vi "Parse Structures.vi"(8 "error in":errorcluster, 11 "ParseGDSII in":refnum<class "ParseGDSII.lvclass">) -> (0 "error out":errorcluster, 2 "Geometric":refnum<class "Geometric.lvclass">[](array[class]), 3 "ParseGDSII out":refnum<class "ParseGDSII.lvclass">)   [LabVIEW 2019, in "ParseGDSII.lvclass"]
uses:
  ParseGDSII.lvclass
  Elements/Geometric.lvclass
  ParseGDSII.lvclass/ParseGDSII.ctl
  Fast Tree/Fast Tree.lvclass
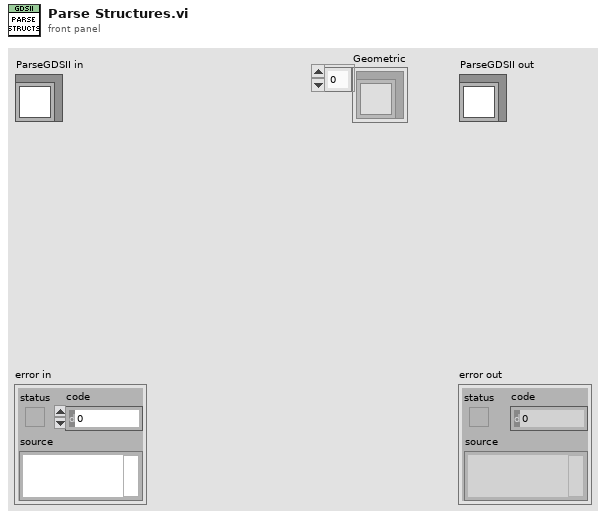
[diagram p1: front panel]
types:
  T1 = cluster{"Record Type":string, "Payload":string, "Parent Index":i32, "First Child Index":i32, "Next Sibling Index":i32}[]
  T2 = cluster{"Record Type":string, "Payload":string, "Parent Index":i32, "First Child Index":i32, "Next Sibling Index":i32}
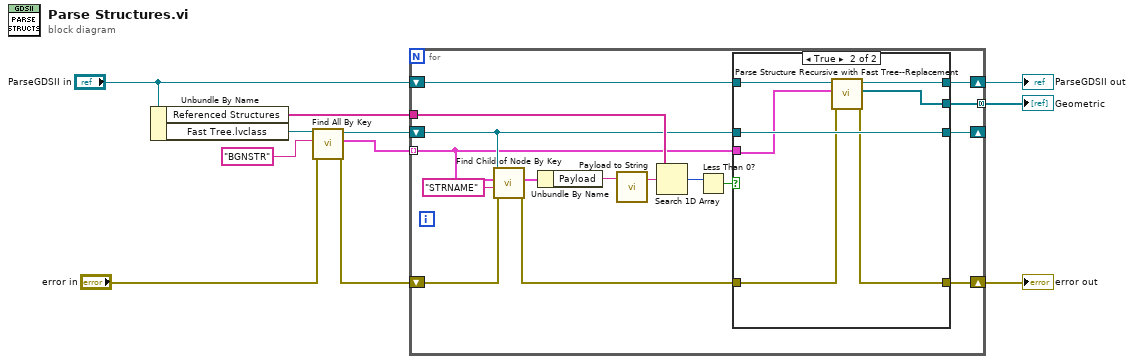
[diagram p0: block diagram]
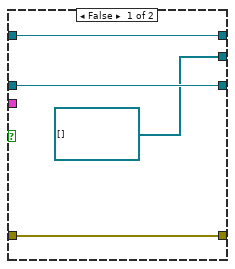
[diagram p2: hidden frame]
diagram:
  n1 = Unbundle By Name("ParseGDSII in") -> ("Referenced Structures"=w3:string[], "Fast Tree.lvclass"=w6:refnum<class "Fast Tree.lvclass">)
  n2 = call "Find All By Key.vi"("error in"="error in", "Key"="BGNSTR", "Fast Tree in"=w6) -> ("error out"=w1:errorcluster, "Found Items"=w4:T1, "Fast Tree out"=w5:refnum<class "Fast Tree.lvclass">)  [unwired: 6 in]
  n3 = for {
    shift-right: [w21] -> _
    shift-left: w5 -> [w20]
    tunnel: w4 -> [w16] mode=indexing
    tunnel: w3 -> [w24]
    tunnel: [w19] -> w8 mode=concatenating
    shift-right: [w17] -> w11
    shift-left: "ParseGDSII in" -> [w18]
    shift-right: [w14] -> w2
    shift-left: w1 -> [w15]
    n4 = call "Find Child of Node By Key.vi"("error in"=w15, "Key"="STRNAME", "Node"=w16, "Fast Tree in"=w20) -> ("error out"=w13:errorcluster, "Child"=w26:T2)  [unwired: 4 in, 2 out]
    n5 = Unbundle By Name(w26) -> ("Payload"=w25:string)
    n6 = call "Payload to String.vi"("Payload"=w25) -> ("String"=w12:string)  [unwired: 2 in]
    n7 = Search 1D Array(1D array=w24, element=w12) -> (index of element=w23:i32)  [unwired: 1 in]
    n8 = Less Than 0?(x=w23) -> (x < 0?=w22:bool)
    n9 = case shown="True" w22 {
      tunnel: [w31 w38] -> w21
      tunnel: w20 -> [w31 w38]
      tunnel: [refnum<class "Geometric.lvclass">[] [] ("Geometric") w32] -> w19
      tunnel: w18 -> [w29 w37]
      tunnel: [w29 w33] -> w17
      tunnel: w16 -> [_ w36]
      tunnel: w13 -> [w28 w35]
      tunnel: [w28 w34] -> w14
      frame False {
      }
      frame True {
        n10 = call "Parse Structure Recursive with Fast Tree--Replacement.vi"("error in"=w35, "Node"=w36, "ParseGDSII in"=w37) -> ("error out"=w34:errorcluster, "Geometric Objects"=w32:refnum<class "Geometric.lvclass">[], "ParseGDSII out"=w33:refnum<class "ParseGDSII.lvclass">)  [unwired: 6 in]
      }
    }
  }
  "error out" <- w2
  "ParseGDSII out" <- w11
  "Geometric" <- w8
